vi "Get RX Message.vi"(8 "error in (no error)":errorcluster, 11 "RxTx in":refnum<class "RxTx.lvclass">) -> (0 "error out":errorcluster, 3 "RxTx out":refnum<class "RxTx.lvclass">)   [LabVIEW 2018, in "RxTx.lvclass"]
uses:
  RxTx.lvclass
  RxTx.lvclass/RxTx.ctl
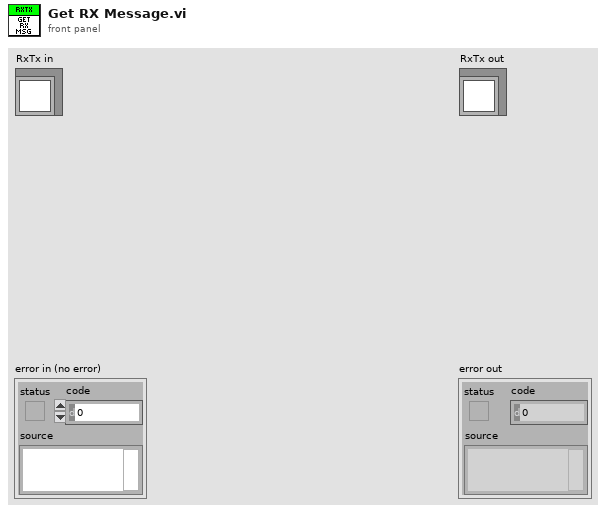
[diagram p1: front panel]
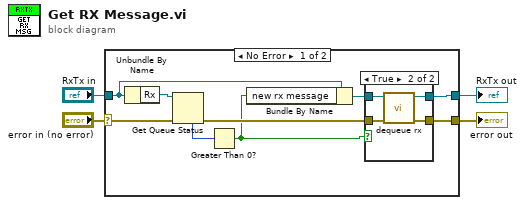
[diagram p0: block diagram]
diagram:
  n1 = case shown="No Error" "error in (no error)" {
    selector: "error in (no error)" -> [w11 w21]
    tunnel: [w9 w21] -> w1
    tunnel: [w13 w20] -> w2
    tunnel: "RxTx in" -> [w7 w20]
    frame No Error {
      n2 = Unbundle By Name(w7) -> ("Rx"=w12:refnum<queue>)
      n3 = Get Queue Status(queue=w12, error in (no error)=w11) -> (error out=w10:errorcluster, # elements in queue=w8:i32)  [unwired: 1 in, 6 out]
      n4 = Greater Than 0?(x=w8) -> (x > 0?=w5:bool)
      n5 = Bundle By Name(cluster=w7, "new rx message"=w5) -> (w6:refnum<class "RxTx.lvclass">)
      n6 = case shown="True" w5 {
        tunnel: w6 -> [w14 w19]
        tunnel: [w14 w18] -> w13
        tunnel: w10 -> [w15 w16]
        tunnel: [w15 w17] -> w9
        frame False {
        }
        frame True {
          n7 = call "dequeue rx.vi"("error in (no error)"=w16, "RxTx in"=w19) -> ("error out"=w17:errorcluster, "RxTx out"=w18:refnum<class "RxTx.lvclass">)  [unwired: 8 in]
        }
      }
    }
    frame Error {
    }
  }
  "error out" <- w1
  "RxTx out" <- w2
